vi "Test_API_Write.vi"() -> ()   [LabVIEW 2021]
doc: "A5a test: Init ? Open ? n × Write_Frame (id, 8 bytes, classic or FD) with a period ? Status ? Close. A Python receiver on CH1 checks the frames."
uses:
  api/CANsub_Channel/CANsub_Channel.lvclass
  common/Typedefs/CANsub_connection.ctl
  common/CANsub_Common.lvlib
  common/Typedefs/CANsub_Bit_Rates.ctl
  api/Typedefs/CANsub_Filter.ctl
  api/CANsub_API.lvlib
  api/Typedefs/CANsub_Read_Mode.ctl
  api/Typedefs/CANsub_Ownership.ctl
  api/Typedefs/CANsub_Config.ctl
  api/Typedefs/CANsub_State.ctl
  common/Typedefs/Bit_Timing.ctl
  api/Typedefs/CANsub_Status.ctl
panel:
  out "error out":errorcluster
  out "status":T1
  in  "period ms":u32=50
  in  "fd":bool
  in  "id":u32=801 format="%.0x"
  in  "n frames":i32=10
  in  "config":T4={"connection"={"host"="192.168.0.49", "channel"=2, "cert path"=path "/home/lvuser/cansub_root_cert.crt"}, "bit rates"={"nominal bit rate"=500000, "nominal sample point"=80.0, "data bit rate"=2000000, "data sample point"=80.0}, "listen only"=FALSE, "filters"=[], "read mode"=enum."Poll", "max bytes per read"=4096, "reader FIFO depth"=0, "reader priority"=0, "ownership"=enum."Direct"} {"filters"."f2" format="%.0x"; "filters"."f1" format="%.0x"}
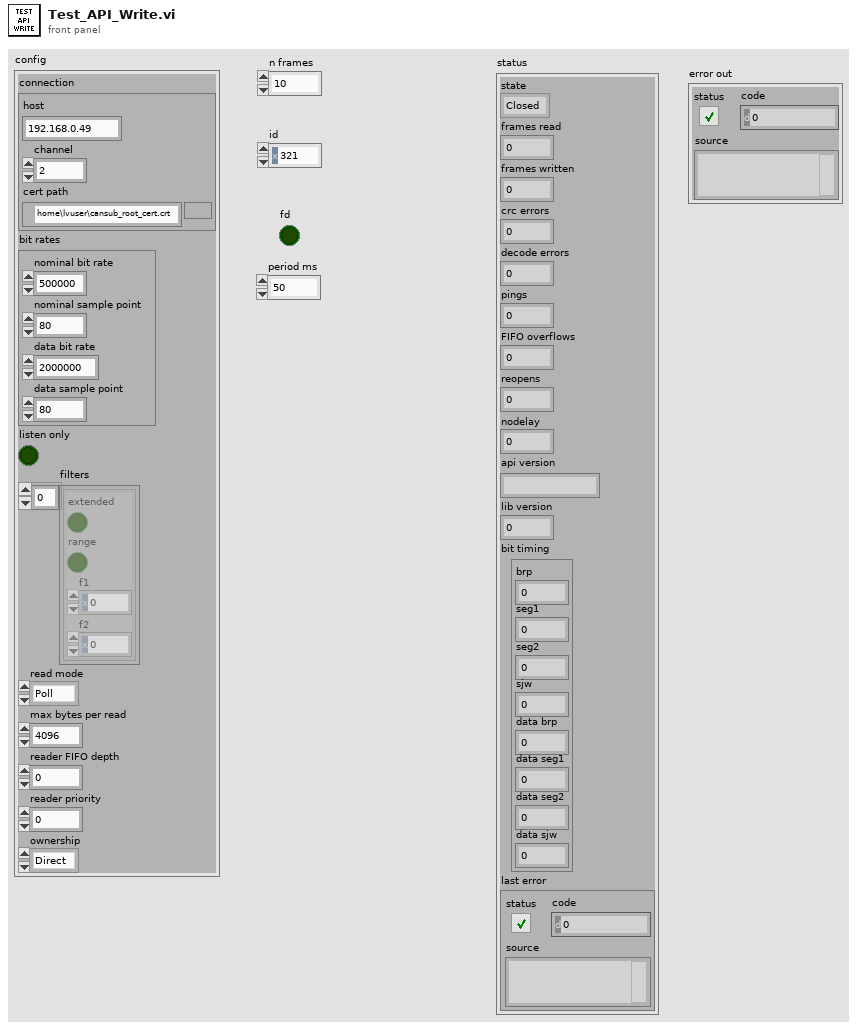
[diagram p1: front panel]
types:
  T1 = typedef "CANsub_API.lvlib/CANsub_Status.ctl" = cluster{"state":T2, "frames read":u32, "frames written":u32, "crc errors":u32, "decode errors":i32, "pings":u32, "FIFO overflows":u32, "reopens":u32, "nodelay":i32, "api version":string, "lib version":u32, "bit timing":T3, "last error":errorcluster}
  T2 = typedef "CANsub_API.lvlib/CANsub_State.ctl" = enum16{"Closed", "Open", "Lost"}
  T3 = typedef "CANsub_Common.lvlib/Bit_Timing.ctl" = cluster{"brp":u16, "seg1":u16, "seg2":u16, "sjw":u16, "data brp":u16, "data seg1":u16, "data seg2":u16, "data sjw":u16}
  T4 = typedef "CANsub_API.lvlib/CANsub_Config.ctl" = cluster{"connection":T5, "bit rates":T6, "listen only":bool, "filters":T7[], "read mode":T8, "max bytes per read":i32, "reader FIFO depth":i32, "reader priority":i32, "ownership":T9}
  T5 = typedef "CANsub_Common.lvlib/CANsub_connection.ctl" = cluster{"host":string, "channel":u8, "cert path":path}
  T6 = typedef "CANsub_Common.lvlib/CANsub_Bit_Rates.ctl" = cluster{"nominal bit rate":u32, "nominal sample point":dbl, "data bit rate":u32, "data sample point":dbl}
  T7 = typedef "CANsub_API.lvlib/CANsub_Filter.ctl" = cluster{"extended":bool, "range":bool, "f1":u32, "f2":u32}
  T8 = typedef "CANsub_API.lvlib/CANsub_Read_Mode.ctl" = enum16{"Poll", "Reader"}
  T9 = typedef "CANsub_API.lvlib/CANsub_Ownership.ctl" = enum16{"Direct", "Shared"}
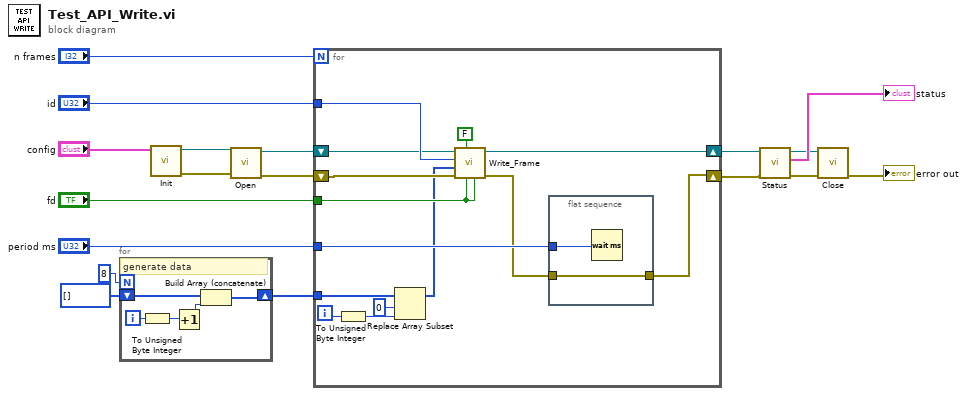
[diagram p0: block diagram]
diagram:
  n1 = for {
    N: 8 -> [_]
    shift-right: [w21] -> w10
    shift-left: u8[] [] -> [w20]
    i -> [w23]
    # "generate data"
    n2 = To Unsigned Byte Integer(number=w23) -> (unsigned 8bit integer=w22:u8)
    n3 = Increment(x=w22) -> (x+1=w19:u8)
    n4 = Build Array (concatenate)(w20, w19) -> (w21:u8[])
  }
  n5 = call "Init.vi"("config"="config") -> ("error out"=w14:errorcluster, "channel out"=w18:refnum<class "CANsub_Channel.lvclass">)  [unwired: 8 in, 1 out]
  n6 = call-dynamic "Open.vi"("error in (no error)"=w14, "channel in"=w18) -> ("error out"=w13:errorcluster, "channel out"=w15:refnum<class "CANsub_Channel.lvclass">)  [unwired: 8 in]
  n7 = for {
    N: "n frames" -> [_]
    shift-right: [w32] -> w3
    shift-left: w15 -> [w36]
    shift-right: [w29] -> w6
    shift-left: w13 -> [w35]
    tunnel: w10 -> [w28]
    tunnel: "id" -> [w37]
    tunnel: "fd" -> [w33]
    tunnel: "period ms" -> [w31]
    i -> [w26]
    n8 = To Unsigned Byte Integer(number=w26) -> (unsigned 8bit integer=w24:u8)
    n9 = Replace Array Subset(array=w28, new element=w24, index=0) -> (w25:u8[])
    n10 = call-dynamic "Write_Frame.vi"("fdf"=w33, "brs"=w33, "ide"=FALSE, "error in (no error)"=w35, "data"=w25, "id"=w37, "channel in"=w36) -> ("error out"=w30:errorcluster, "channel out"=w32:refnum<class "CANsub_Channel.lvclass">)  [unwired: 3 in]
    n11 = flat-sequence {
      tunnel: w31 -> [w39]
      tunnel: w30 -> [w38]
      tunnel: [w38] -> w29
      frame #0 {
        n12 = Wait (ms)(milliseconds to wait=w39) -> ()  [unwired: 1 out]
      }
    }
  }
  n13 = call-dynamic "Status.vi"("error in (no error)"=w6, "channel in"=w3) -> ("error out"=w5:errorcluster, "status"=→"status":T1, "channel out"=w2:refnum<class "CANsub_Channel.lvclass">)  [unwired: 7 in]
  n14 = call-dynamic "Close.vi"("error in (no error)"=w5, "channel in"=w2) -> ("error out"=→"error out":errorcluster)  [unwired: 8 in, 1 out]
